vi "Motor Test Bench.vi"() -> ()   [LabVIEW 2021]
uses:
  Modbus_TCP/Modbus_TCP.lvclass
  C:/Users/lincoln.lucio/Documents/Lincoln/Documentos Pessoais/meus docs/Projetos pessoais/Projeto Sciranda/projeto_versioned/sciranda/Modbus_Master/Modbus_Master.lvclass
  Modbus_AI/Modbus_AI.lvclass
  C:/Users/lincoln.lucio/Documents/Lincoln/Documentos Pessoais/meus docs/Projetos pessoais/Projeto Sciranda/projeto_versioned/sciranda/AnalogInput/AnalogInput.lvclass
  Modbus_AO/Modbus_AO.lvclass
  C:/Users/lincoln.lucio/Documents/Lincoln/Documentos Pessoais/meus docs/Projetos pessoais/Projeto Sciranda/projeto_versioned/sciranda/AnalogOutput/AnalogOutput.lvclass
  Motor/Motor.lvclass
  Modbus_TCP/Modbus_TCP.lvclass/Modbus_TCP.ctl
  Modbus_AI/Modbus_AI.lvclass/Modbus_AI.ctl
  Modbus_AO/Modbus_AO.lvclass/Modbus_AO.ctl
  Motor/Motor.lvclass/Motor.ctl
  Modbus_Master/Modbus_Master.lvclass
  Modbus_TCP/Accessor VIs/Write Port.vi
  Modbus_AI/Accessor VIs/Write Modbus_Master.lvclass.vi
  Modbus_AI/Accessor VIs/Read Modbus_Master.lvclass.vi
  Modbus_AI/Accessor VIs/Write Register Address.vi
  Modbus_AO/Accessor VIs/Write Modbus_Master.lvclass.vi
  Modbus_AO/Accessor VIs/Write Register Address.vi
  Modbus_AO/Accessor VIs/Read Modbus_Master.lvclass.vi
panel:
  in  "Enum":enum16{"DAQNavi", "Modbus_TCP", "Modbus_RTU"}(ring)
  in  "stop":bool
  out "Actual Speed":dbl
  in  "Motor Control":dbl
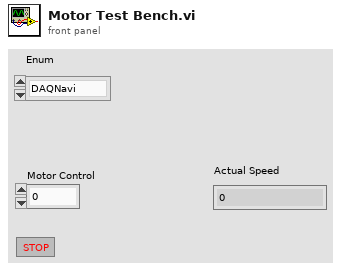
[diagram p1: front panel]
types:
  T1 = typedef "Device Context Cluster.ctl" = cluster{"Motor in":refnum<class "Motor.lvclass">, "Elevator.lvclass":refnum<class "Elevator.lvclass">}
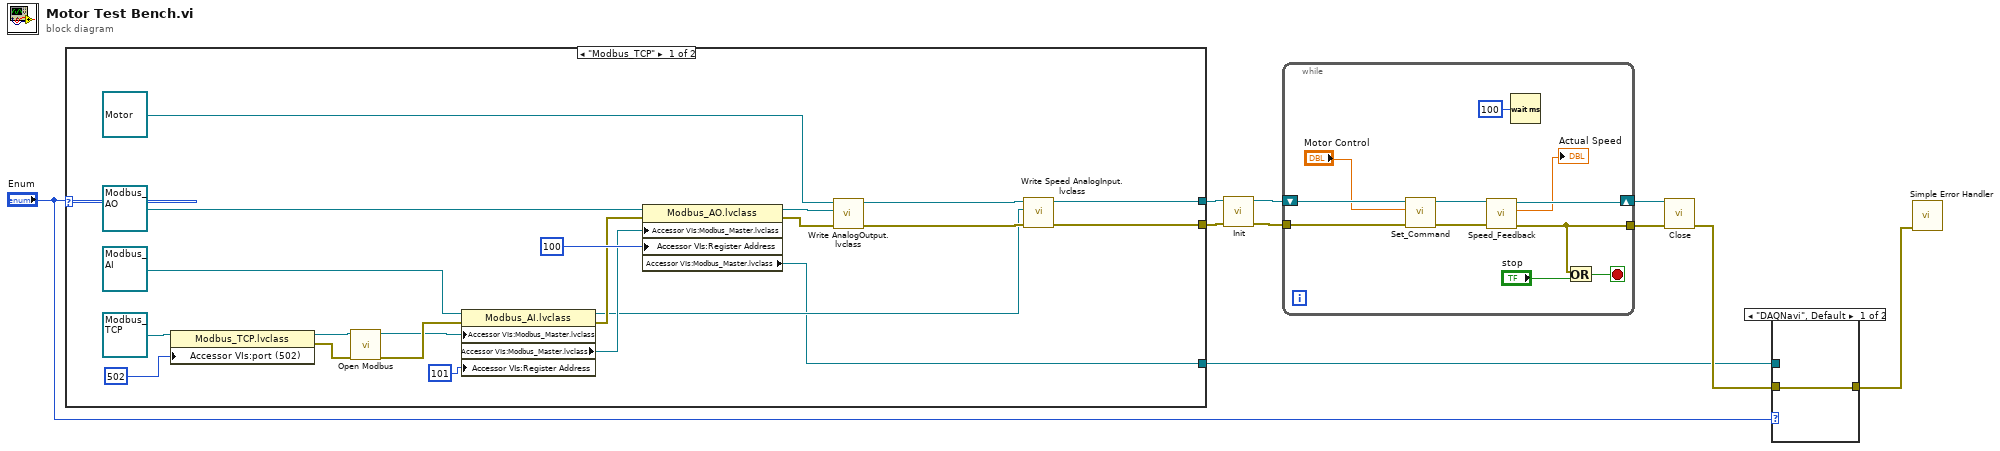
[diagram p0: block diagram]
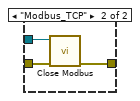
[diagram p2: hidden frame]
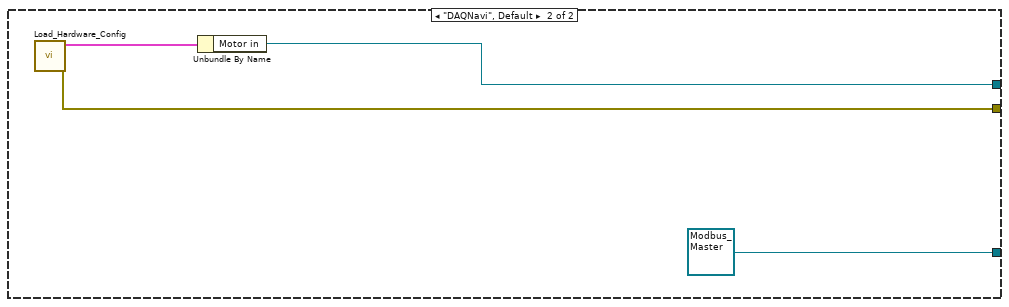
[diagram p3: hidden frame]
diagram:
  n1 = case shown="\"Modbus_TCP\"" "Enum" {
    tunnel: [w19 w35] -> w10
    tunnel: [w18 w34] -> w7
    tunnel: [w11 refnum<class "Modbus_Master.lvclass"> refnum ("Accessor VIs:Modbus_Master.lvclass")] -> w2
    frame "Modbus_TCP" {
      n2 = property class="Modbus_TCP.lvclass"(reference=refnum<class "Modbus_TCP.lvclass"> refnum ("Modbus_TCP.lvclass"), "Accessor VIs:port (502)"=u16 502 ("port (502)")) -> (reference out=w13:refnum<class "Modbus_TCP.lvclass">, error out=w15:errorcluster)  [unwired: 1 in]
      n3 = call-dynamic "Open Modbus.vi"("error in (no error)"=w15, "Modbus_TCP in"=w13) -> ("error out"=w14:errorcluster, "Modbus_TCP out"=w12:refnum<class "Modbus_TCP.lvclass">)  [unwired: 8 in]
      n4 = property class="Modbus_AI.lvclass"(reference=refnum<class "Modbus_AI.lvclass"> refnum ("Modbus_AI.lvclass"), error in=w14, "Accessor VIs:Modbus_Master.lvclass"=w12, "Accessor VIs:Register Address"=u16 101 ("Register Address")) -> (reference out=w17:refnum<class "Modbus_AI.lvclass">, error out=w25:errorcluster, "Accessor VIs:Modbus_Master.lvclass"=w26:refnum<class "Modbus_Master.lvclass">)
      n5 = property class="Modbus_AO.lvclass"(reference=refnum<class "Modbus_AO.lvclass"> refnum ("Modbus_AO.lvclass"), error in=w25, "Accessor VIs:Modbus_Master.lvclass"=w26, "Accessor VIs:Register Address"=u16 100 ("Register Address")) -> (reference out=w23:refnum<class "Modbus_AO.lvclass">, error out=w22:errorcluster, "Accessor VIs:Modbus_Master.lvclass"=w11:refnum<class "Modbus_Master.lvclass">)
      n6 = call "Write AnalogOutput.lvclass.vi"("error in (no error)"=w22, "AnalogOutput.lvclass"=w23, "Motor in"=refnum<class "Motor.lvclass"> refnum) -> ("error out"=w20:errorcluster, "Motor out"=w21:refnum<class "Motor.lvclass">)  [unwired: 7 in]
      n7 = call "Write Speed AnalogInput.lvclass.vi"("error in (no error)"=w20, "AnalogInput.lvclass"=w17, "Motor in"=w21) -> ("error out"=w19:errorcluster, "Motor out"=w18:refnum<class "Motor.lvclass">)  [unwired: 7 in]
    }
    frame "DAQNavi", Default {
      n8 = call "Load_Hardware_Config.vi"() -> ("error out"=w35:errorcluster, "Device Context Cluster"=w33:T1)  [unwired: 10 in]
      n9 = Unbundle By Name(w33) -> ("Motor in"=w34:refnum<class "Motor.lvclass">)
    }
  }
  n10 = call "Init.vi"("error in (no error)"=w10, "Motor in"=w7) -> ("error out"=w9:errorcluster, "Motor out"=w8:refnum<class "Motor.lvclass">)  [unwired: 8 in]
  n11 = while {
    shift-right: [w38] -> w4
    shift-left: w8 -> [w43]
    tunnel: w9 -> [w41]
    tunnel: [w36] -> w6
    stop <- w44 stop-if-true
    n12 = call "Set_Command.vi"("error in (no error)"=w41, "Motor Control"="Motor Control", "Motor in"=w43) -> ("error out"=w39:errorcluster, "Motor out"=w40:refnum<class "Motor.lvclass">)  [unwired: 7 in]
    n13 = call "Speed_Feedback.vi"("error in (no error)"=w39, "Motor in"=w40) -> ("error out"=w36:errorcluster, "Actual Speed"=→"Actual Speed":dbl, "Motor out"=w38:refnum<class "Motor.lvclass">)  [unwired: 7 in]
    n14 = Wait (ms)(milliseconds to wait=u32 100) -> ()  [unwired: 1 out]
    n15 = Or(x=w36, y="stop") -> (x .or. y?=w44:bool)
  }
  n16 = call "Close.vi"("error in (no error)"=w6, "Motor in"=w4) -> ("error out"=w5:errorcluster)  [unwired: 8 in, 1 out]
  n17 = case shown="\"DAQNavi\", Default" "Enum" {
    tunnel: w5 -> [w47 w50]
    tunnel: w2 -> [_ w49]
    tunnel: [w47 w48] -> w3
    frame "DAQNavi", Default {
    }
    frame "Modbus_TCP" {
      n18 = call "Close Modbus.vi"("error in (no error)"=w50, "Modbus_Master in"=w49) -> ("error out"=w48:errorcluster)  [unwired: 8 in, 1 out]
    }
  }
  n19 = call <vilib>:"Simple Error Handler.vi"("error in (no error)"=w3) -> ()  [unwired: 4 in, 5 out]
